vi "Create_ini_file.vi"(7 "Name":string, 8 "error in (no error)":errorcluster) -> (0 "error out":errorcluster, 3 "path":path)   [LabVIEW 2021]
uses:
  <vilib>/Utility/config.llb/NI_LVConfig.lvlib
panel:
  out "appended path":path
  out "concatenated string":string
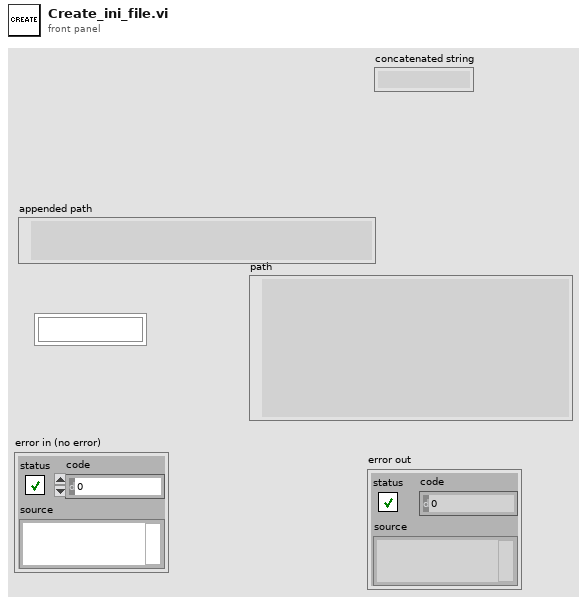
[diagram p1: front panel]
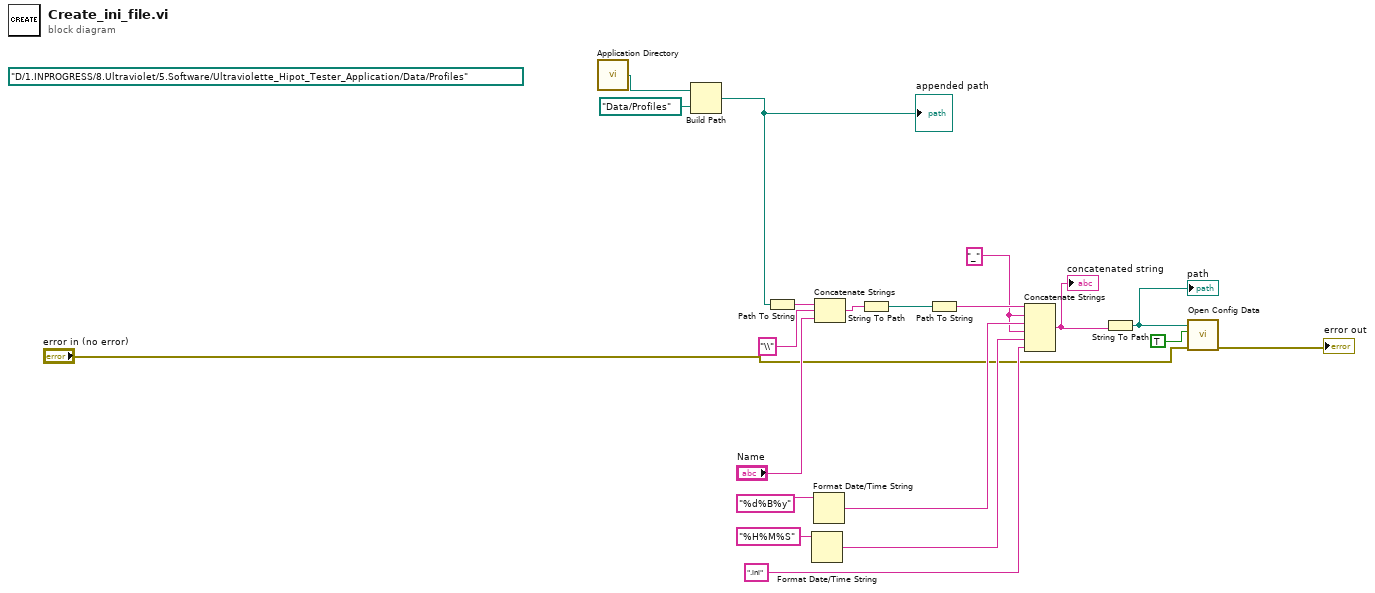
[diagram p0: block diagram]
diagram:
  (unwired) path "D:/1.INPROGRESS/8.Ultraviolet/5.Software/Ultraviolette_Hipot_Tester_Application/Data/Profiles" ("configuration file path")
  w7 = "_" ("string")
  n1 = call <vilib>:"Application Directory.vi"() -> ("Application Directory"=w17:path)
  n2 = Build Path(base path=w17, name or relative path=path "Data/Profiles") -> (appended path=w2:path)
  "appended path" <- w2
  n3 = Path To String(path=w2) -> (string=w5:string)
  n4 = Format Date/Time String(time format string (%c)="%H%M%S") -> (date/time string=w13:string)  [unwired: 2 in]
  n5 = Format Date/Time String(time format string (%c)="%d%B%y") -> (date/time string=w14:string)  [unwired: 2 in]
  n6 = Concatenate Strings(w5, "\\" ("string"), "Name") -> (w4:string)
  n7 = String To Path(string=w4) -> (path=w16:path)
  n8 = Path To String(path=w16) -> (string=w15:string)
  n9 = Concatenate Strings(w15, w7, w14, w7, w13, ".ini" ("string")) -> (w12:string)
  "concatenated string" <- w12
  n10 = String To Path(string=w12) -> (path=w11:path)
  "path" <- w11
  n11 = call <vilib>:"Open Config Data.vi"("error in (no error)"="error in (no error)", "create file if necessary (T)"=TRUE, "configuration file path"=w11) -> ("error out"=→"error out":errorcluster)  [unwired: 6 in, 2 out]
